vi "take cabinet.vi"(2 "error in (no error)":errorcluster, 3 "高度":i32) -> (0 "error out":errorcluster)   [LabVIEW 2019]
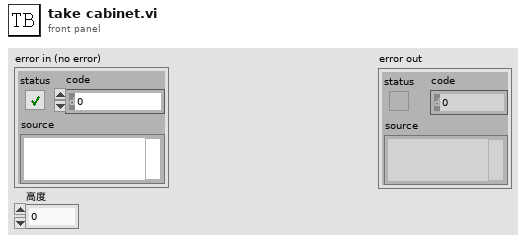
[diagram p1: front panel]
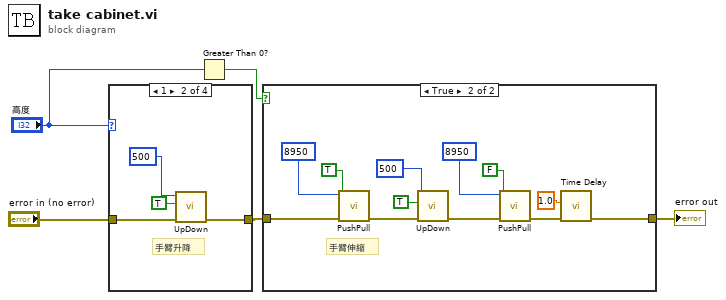
[diagram p0: block diagram]
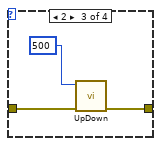
[diagram p4: hidden frame]
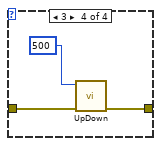
[diagram p5: hidden frame]
diagram:
  n1 = case shown="1" "高度" {
    tunnel: "error in (no error)" -> [w6 w10 w13 w16]
    tunnel: [w6 w8 w11 w14] -> w4
    frame 0, Default {
    }
    frame 1 {
      # "手臂升降"
      n2 = call "UpDown.vi"("error in (no error)"=w10, "轉向"=TRUE, "距離"=500) -> ("error out"=w8:errorcluster)  [unwired: 7 in, 1 out]
    }
    frame 2 {
      n3 = call "UpDown.vi"("error in (no error)"=w13, "距離"=500) -> ("error out"=w11:errorcluster)  [unwired: 8 in, 1 out]
    }
    frame 3 {
      n4 = call "UpDown.vi"("error in (no error)"=w16, "距離"=500) -> ("error out"=w14:errorcluster)  [unwired: 8 in, 1 out]
    }
  }
  n5 = Greater Than 0?(x="高度") -> (x > 0?=w2:bool)
  n6 = case shown="True" w2 {
    tunnel: w4 -> [w17 w27]
    tunnel: [w17 w18] -> w3
    frame False {
    }
    frame True {
      # "手臂伸縮"
      n7 = call "PushPull.vi"("error in (no error)"=w27, "轉向"=TRUE, "距離"=8950) -> ("error out"=w24:errorcluster)  [unwired: 7 in, 1 out]
      n8 = call "UpDown.vi"("error in (no error)"=w24, "轉向"=TRUE, "距離"=500) -> ("error out"=w21:errorcluster)  [unwired: 7 in, 1 out]
      n9 = call "PushPull.vi"("error in (no error)"=w21, "轉向"=FALSE, "距離"=8950) -> ("error out"=w19:errorcluster)  [unwired: 7 in, 1 out]
      n10 = call "Time Delay"("error in (no error)"=w19, "Delay Time (s)"=1.0) -> ("error out"=w18:errorcluster)  [unwired: 9 in]
    }
  }
  "error out" <- w3
